vi "MQTT Connect - Init.vi"(0 "MQTT ref in":T2, 5 "Keep Alive":u16, 7 "Clean start":bool, 9 "Connect Properties":T1[](array[typedef]) {"Property" items=[" Session Expiry Interval           "=17, " Authentication Method             "=21, " Authentication Data               "=22, " Request Problem Information       "=23, " Request Response Information      "=25, " Receive Maximum                   "=33, " Topic Alias Maximum               "=34, " User Property                     "=38, " Maximum Packet Size               "=39]}, 11 "error in (no error)":errorcluster) -> (4 "MQTT ref out":T2, 15 "error out":errorcluster)   [LabVIEW 2019, in "KoRE-MQTT.lvlib"]
doc: "This VI initializes all session parameters for a new client connection. It applies client-requested CONNECT properties and therequested Keep Alive and sets server-controlled parameters to their default values. \n\nThe server may override client-requested or server-default values by returning one or more CONNACK properties during the final connection handshake. The MQTT specification does not require the server to confirm requested or default values; the server sends CONNACK properties only when it rejects or changes a value. Because CONNACK can change session parameters after this VI runs, the VI initializes the runtime with the client-requested values when present and updates other values according to defaults as according to the MQTT v5 standard.\n\nOn CONNACK receipt the code will inspect CONNACK properties and update session state for any rejected or modified parameters. \n\nCopyright (c) 2025 KoRElibs.com\nSPDX-License-Identifier: EUPL-1.2\n\nThis VI is licensed under the European Union Public License (EUPL) Version 1.2. You may use this VI unmodified in proprietary works. If you distribute a modified version of this file, the modified file must be released under the EUPL-1.2. Full license: https://joinup.ec.europa.eu/asset/eupl/eupl/1.2/"
uses:
  KoRE-MQTT.lvlib
  Public/TypeDefs/MQTT Client Session.ctl
  Public/TypeDefs/MQTT Property - CONNECT.ctl
  Public/TypeDefs/MQTT Version.ctl
  TypeDefs/MQTT Subscription - Info.ctl
  Public/TypeDefs/MQTT Property Type.ctl
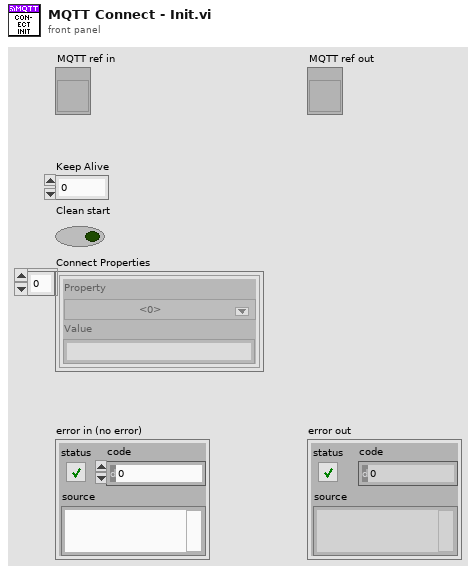
[diagram p1: front panel]
types:
  T1 = typedef "KoRE-MQTT.lvlib/MQTT Property - CONNECT.ctl" = cluster{"Property":u8, "Value":string}
  T2 = typedef "KoRE-MQTT.lvlib/MQTT Client Session.ctl" = refnum<vi>
  T3 = typedef "KoRE-MQTT.lvlib/MQTT Version.ctl" = u16
  T4 = typedef "KoRE-MQTT.lvlib/MQTT Client Session - Data.ctl" = cluster{"TCP ref":refnum<k5>, "Next Packet Id":u16, "Version":u8, "Host":string, "Port":u16, "Ping Delta":u32, "Username":string, "Password":string, "Will QoS":u8, "Will Retain":bool, "Will Topic":string, "Will Payload":string, "TCP Timeout":i32, "Semaphore":T5, "In-Flight Messages":variant, "Close":bool, "Last Send":u32, "Keep Alive":u16, "Last Ping RTT":u32, "Last Ping":u32, "Will Properties":T6[], "Session Expiry Interval":u32, "Maximum QoS":u8, "Retain Available":bool, "Server Maximum Packet Size":u32, "Client Identifier":string, "Server Topic Alias Maximum":u16, "Wildcard Subscription Available":bool, "Subscription Identifier Available":bool, "Shared Subscription Available":bool, "Connect Properties":T1[], "Client Maximum Packet Size":u32, "Client Topic Alias Maximum":u16, "Server Receive Maximum":u16, "Client Receive Maximum":u16, "TLS cfg":refnum<k36>, "Subscriptions":T7[]}
  T5 = typedef "Semaphore RefNum" = refnum<k1>
  T6 = typedef "KoRE-MQTT.lvlib/MQTT Property - Will.ctl" = cluster{"Property":u8, "Value":string}
  T7 = typedef "KoRE-MQTT.lvlib/MQTT Subscription - Info.ctl" = cluster{"Packet Id":u16, "Index":u16, "Identifier":u32, "QoS":u8, "Topic Filter":string, "Reason Code":u8, "Reason String":string, "Granted":bool}
  T8 = typedef "KoRE-MQTT.lvlib/MQTT Property Type.ctl" = u8
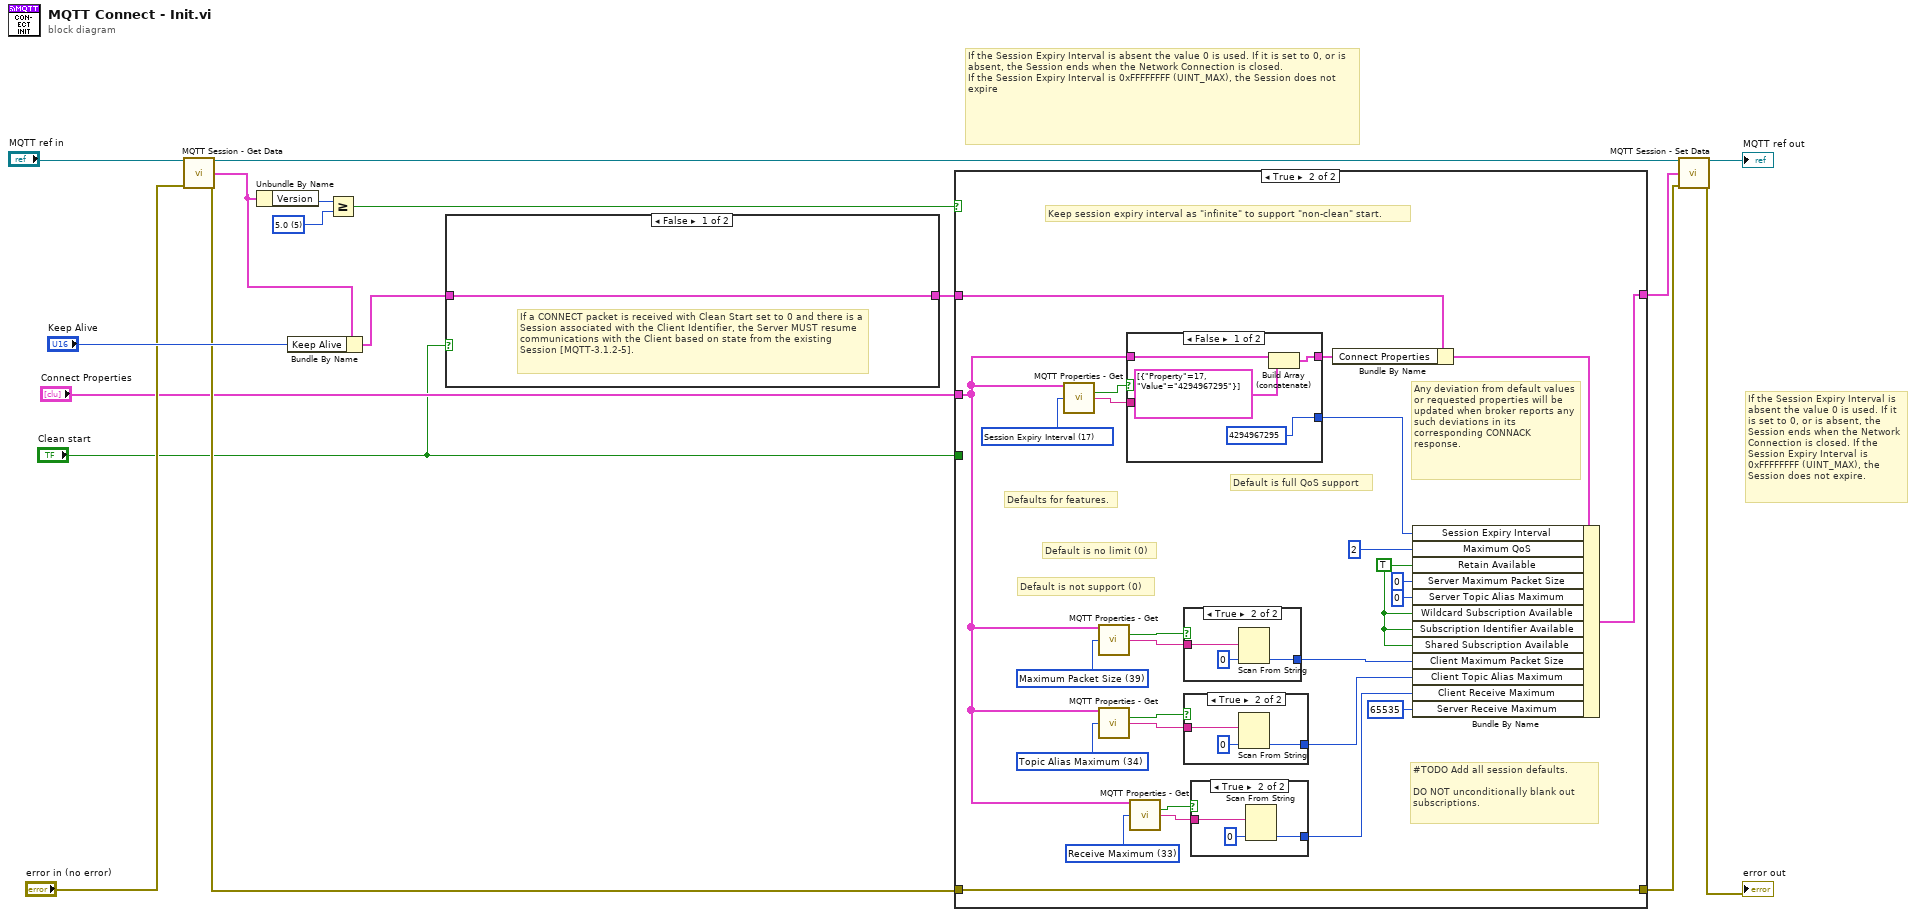
[diagram p0: block diagram]
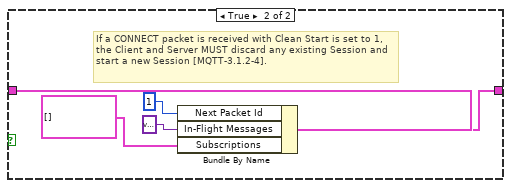
[diagram p2: hidden frame]
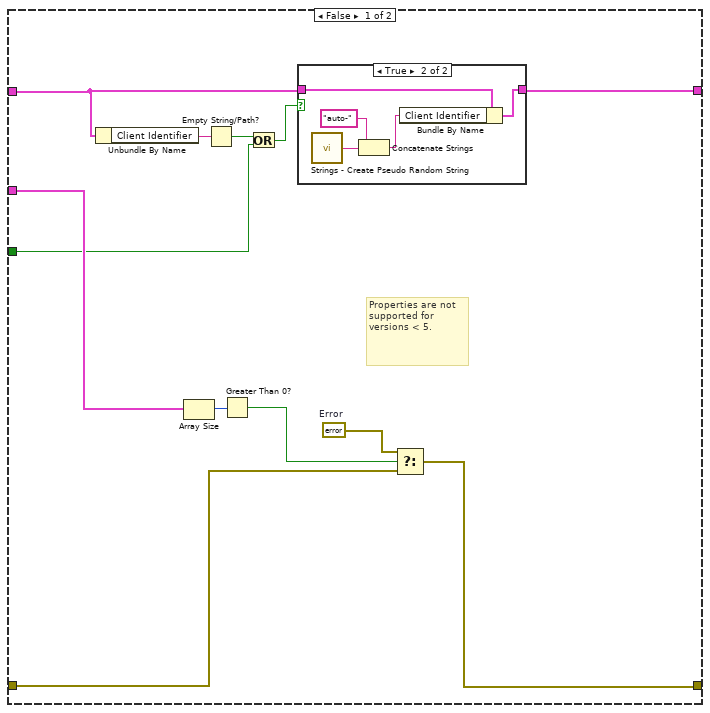
[diagram p3: hidden frame]
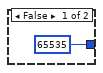
[diagram p5: hidden frame]
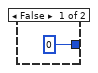
[diagram p6: hidden frame]
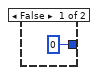
[diagram p7: hidden frame]
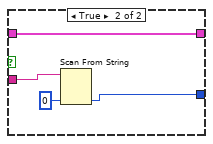
[diagram p8: hidden frame]
diagram:
  w9 = T3 5 items=["3.11"=4, "5.0"=5] ("y")
  # "If the Session Expiry Interval is absent the value 0 is used. If it is set to 0, or is absent, the Session ends when the Network Connection is closed.\nIf the Session Expiry Interval is 0xFFFFFFFF (UINT_MAX), the Session does not expire"
  # "If the Session Expiry Interval is absent the value 0 is used. If it is set to 0, or is absent, the Session ends when the Network Connection is closed. If the Session Expiry Interval is 0xFFFFFFFF (UINT_MAX), the Session does not expire."
  n1 = call "MQTT Session - Get Data.vi"("mqtt ref in"="MQTT ref in", "error in"="error in (no error)") -> ("mqtt ref out"=w11:T2, "mqtt ref data"=w12:T4, "error out"=w5:errorcluster)  [unwired: 11 in]
  n2 = Unbundle By Name(w12) -> ("Version"=w10:u8)
  n3 = Bundle By Name(cluster=w12, "Keep Alive"="Keep Alive") -> (w3:T4)
  n4 = Greater Or Equal?(x=w10, y=w9) -> (x >= y?=w13:bool)
  n5 = case shown="False" "Clean start" {
    tunnel: [w18 w22] -> w2
    tunnel: w3 -> [w18 w23]
    frame False {
      # "If a CONNECT packet is received with Clean Start set to 0 and there is a Session associated with the Client Identifier, the Server MUST resume communications with the Client based on state from the existing Session [MQTT-3.1.2-5]."
    }
    frame True {
      # "If a CONNECT packet is received with Clean Start is set to 1, the Client and Server MUST discard any existing Session and start a new Session [MQTT-3.1.2-4]."
      n6 = Bundle By Name(cluster=w23, "Next Packet Id"=u16 1, "In-Flight Messages"=variant, "Subscriptions"=T7[] []) -> (w22:T4)
    }
  }
  n7 = case shown="True" w13 {
    tunnel: [w34 w68] -> w8
    tunnel: w5 -> [w33 w68]
    tunnel: w2 -> [w31 w67]
    tunnel: [w30 w63] -> w17
    tunnel: "Connect Properties" -> [w25 w42]
    tunnel: "Clean start" -> [w24 _]
    frame False {
      w35 = errorcluster {"status"=TRUE, "code"=5000, "source"="MQTT Properties are only supported from MQTT protocol v 5.0."}  # Error
      # "Properties are not supported for versions < 5."
      n8 = Unbundle By Name(w31) -> ("Client Identifier"=w32:string)
      n9 = Array Size(array=w25) -> (size(s)=w28:i32)
      n10 = Empty String/Path?(string/path=w32) -> (empty?=w29:bool)
      n11 = Greater Than 0?(x=w28) -> (x > 0?=w27:bool)
      n12 = Or(x=w29, y=w24) -> (x .or. y?=w26:bool)
      n13 = case shown="True" w26 {
        tunnel: w31 -> [w36 w41]
        tunnel: [w36 w40] -> w30
        frame False {
        }
        frame True {
          n14 = call "Strings - Create Pseudo Random String.vi"() -> ("Pseudorandom String"=w39:string)  [unwired: 9 in]
          n15 = Concatenate Strings("auto-" ("string"), w39) -> (w37:string)
          n16 = Bundle By Name(cluster=w41, "Client Identifier"=w37) -> (w40:T4)
        }
      }
      n17 = Select(t=w35, s=w27, f=w33) -> (s? t:f=w34:errorcluster)
    }
    frame True {
      w47 = T8 33 items=["Payload Format Indicator"=1, "Message Expiry Interval"=2, "Content Type"=3, "Response Topic"=8, "Correlation Data"=9, "Subscription Identifier"=11, "Session Expiry Interval"=17, "Assigned Client Identifier"=18, "Server Keep Alive"=19, "Authentication Method"=21, "Authentication Data"=22, "Request Problem Information"=23, "Will Delay Interval"=24, "Request Response Information"=25, "Response Information"=26, "Server Reference"=28, "Reason String"=31, "Receive Maximum"=33, "Topic Alias Maximum"=34, "Topic Alias"=35, "Maximum QoS"=36, "Retain Available"=37, "User Property"=38, "Maximum Packet Size"=39, "Wildcard Subscription Available"=40, "Subscription Identifier Available"=41, "Shared Subscription Available"=42] ("MQTT Property Type")
      w55 = T8 34 items=["Payload Format Indicator"=1, "Message Expiry Interval"=2, "Content Type"=3, "Response Topic"=8, "Correlation Data"=9, "Subscription Identifier"=11, "Session Expiry Interval"=17, "Assigned Client Identifier"=18, "Server Keep Alive"=19, "Authentication Method"=21, "Authentication Data"=22, "Request Problem Information"=23, "Will Delay Interval"=24, "Request Response Information"=25, "Response Information"=26, "Server Reference"=28, "Reason String"=31, "Receive Maximum"=33, "Topic Alias Maximum"=34, "Topic Alias"=35, "Maximum QoS"=36, "Retain Available"=37, "User Property"=38, "Maximum Packet Size"=39, "Wildcard Subscription Available"=40, "Subscription Identifier Available"=41, "Shared Subscription Available"=42] ("MQTT Property Type")
      w61 = T8 39 items=["Payload Format Indicator"=1, "Message Expiry Interval"=2, "Content Type"=3, "Response Topic"=8, "Correlation Data"=9, "Subscription Identifier"=11, "Session Expiry Interval"=17, "Assigned Client Identifier"=18, "Server Keep Alive"=19, "Authentication Method"=21, "Authentication Data"=22, "Request Problem Information"=23, "Will Delay Interval"=24, "Request Response Information"=25, "Response Information"=26, "Server Reference"=28, "Reason String"=31, "Receive Maximum"=33, "Topic Alias Maximum"=34, "Topic Alias"=35, "Maximum QoS"=36, "Retain Available"=37, "User Property"=38, "Maximum Packet Size"=39, "Wildcard Subscription Available"=40, "Subscription Identifier Available"=41, "Shared Subscription Available"=42] ("MQTT Property Type")
      w49 = TRUE ("Retain Available")
      w64 = T8 17 items=["Payload Format Indicator"=1, "Message Expiry Interval"=2, "Content Type"=3, "Response Topic"=8, "Correlation Data"=9, "Subscription Identifier"=11, "Session Expiry Interval"=17, "Assigned Client Identifier"=18, "Server Keep Alive"=19, "Authentication Method"=21, "Authentication Data"=22, "Request Problem Information"=23, "Will Delay Interval"=24, "Request Response Information"=25, "Response Information"=26, "Server Reference"=28, "Reason String"=31, "Receive Maximum"=33, "Topic Alias Maximum"=34, "Topic Alias"=35, "Maximum QoS"=36, "Retain Available"=37, "User Property"=38, "Maximum Packet Size"=39, "Wildcard Subscription Available"=40, "Subscription Identifier Available"=41, "Shared Subscription Available"=42] ("MQTT Property Type")
      # "#TODO Add all session defaults.\n\nDO NOT unconditionally blank out\nsubscriptions."
      # "Keep session expiry interval as \"infinite\" to support \"non-clean\" start."
      # "Any deviation from default values or requested properties will be updated when broker reports any such deviations in its corresponding CONNACK response."
      # "Default is not support (0)"
      # "Default is no limit (0)"
      # "Defaults for features."
      # "Default is full QoS support"
      n18 = call "MQTT Properties - Get.vi"("MQTT Properties"=w42, "MQTT Property Type"=w64) -> ("Found"=w59:bool, "Value"=w66:string)  [unwired: 11 in, 1 out]
      n19 = call "MQTT Properties - Get.vi"("MQTT Properties"=w42, "MQTT Property Type"=w61) -> ("Found"=w57:bool, "Value"=w60:string)  [unwired: 11 in, 1 out]
      n20 = call "MQTT Properties - Get.vi"("MQTT Properties"=w42, "MQTT Property Type"=w55) -> ("Found"=w53:bool, "Value"=w54:string)  [unwired: 11 in, 1 out]
      n21 = case shown="False" w59 {
        tunnel: w66 -> [_ w88]
        tunnel: [u32 4294967295 ("default value 14") w86] -> w58
        tunnel: [w83 w85] -> w48
        tunnel: w42 -> [w81 w85]
        frame False {
          n22 = Build Array (concatenate)(w81, T1[] [{"Property"=17, "Value"="4294967295"}] ("array")) -> (w83:T1[])
        }
        frame True {
          n23 = Scan From String(input string=w88, default 1=u32 0 ("default value 14")) -> (output 1=w86:u32)  [unwired: 3 in, 3 out]
        }
      }
      n24 = call "MQTT Properties - Get.vi"("MQTT Properties"=w42, "MQTT Property Type"=w47) -> ("Found"=w45:bool, "Value"=w46:string)  [unwired: 11 in, 1 out]
      n25 = case shown="True" w57 {
        tunnel: w60 -> [_ w79]
        tunnel: [u32 0 ("default value 14") w78] -> w56
        frame False {
        }
        frame True {
          n26 = Scan From String(input string=w79, default 1=u32 0 ("default value 14")) -> (output 1=w78:u32)  [unwired: 3 in, 3 out]
        }
      }
      n27 = case shown="True" w53 {
        tunnel: w54 -> [_ w75]
        tunnel: [u16 0 ("default value 14") w74] -> w52
        frame False {
        }
        frame True {
          n28 = Scan From String(input string=w75, default 1=u16 0 ("default value 14")) -> (output 1=w74:u16)  [unwired: 3 in, 3 out]
        }
      }
      n29 = case shown="True" w45 {
        tunnel: w46 -> [_ w71]
        tunnel: [u16 65535 ("Client Receive Maximum") w70] -> w44
        frame False {
        }
        frame True {
          n30 = Scan From String(input string=w71, default 1=u16 0 ("default value 14")) -> (output 1=w70:u16)  [unwired: 3 in, 3 out]
        }
      }
      n31 = Bundle By Name(cluster=w67, "Connect Properties"=w48) -> (w65:T4)
      n32 = Bundle By Name(cluster=w65, "Session Expiry Interval"=w58, "Maximum QoS"=u8 2, "Retain Available"=w49, "Server Maximum Packet Size"=u32 0, "Server Topic Alias Maximum"=u16 0, "Wildcard Subscription Available"=w49, "Subscription Identifier Available"=w49, "Shared Subscription Available"=w49, "Client Maximum Packet Size"=w56, "Client Topic Alias Maximum"=w52, "Client Receive Maximum"=w44, "Server Receive Maximum"=u16 65535) -> (w63:T4)
    }
  }
  n33 = call "MQTT Session - Set Data.vi"("mqtt ref in"=w11, "mqtt ref data"=w17, "error in"=w8) -> ("mqtt ref out"=→"MQTT ref out":T2, "error out"=→"error out":errorcluster)  [unwired: 11 in]
